vi "DAQ_Main.vi"() -> ()   [LabVIEW 2026]
panel:
  out "samples_logged":dbl
  out "overpressure":bool
  out "pressure_chart":dbl(graph)
  out "pressure_bar":dbl
  in  "stop_acquisition":bool
  in  "start_acquisition":bool
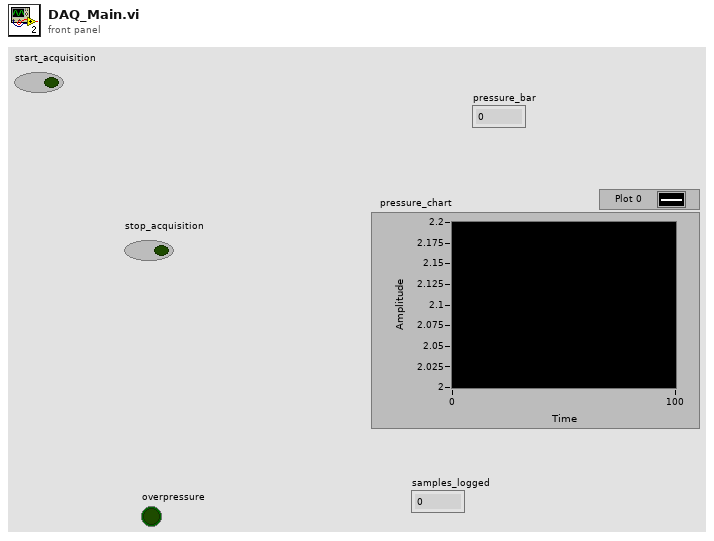
[diagram p1: front panel]
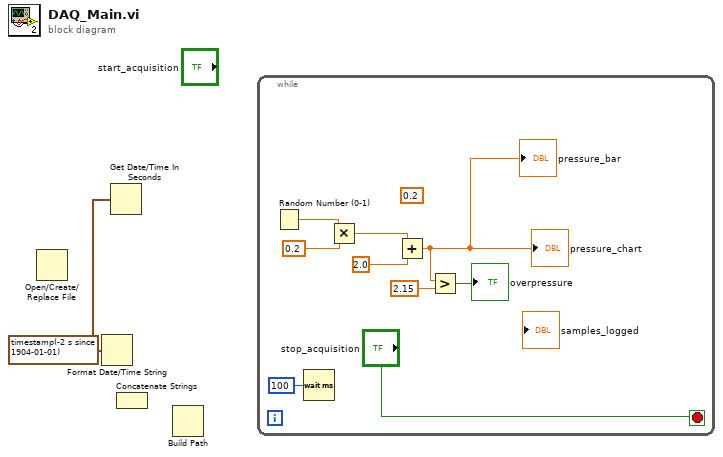
[diagram p0: block diagram]
diagram:
  (unwired) timestamp(-2 s since 1904-01-01) ("time stamp")
  n1 = Open/Create/Replace File() -> ()  [unwired: 6 in, 3 out]
  n2 = Get Date/Time In Seconds() -> (seconds since 1Jan1904=w1:timestamp)
  n3 = Format Date/Time String(seconds (now)=w1) -> ()  [unwired: 2 in, 1 out]
  n4 = Concatenate Strings() -> ()  [unwired: 2 in, 1 out]
  n5 = Build Path() -> ()  [unwired: 2 in, 1 out]
  n6 = while {
    stop <- "stop_acquisition" stop-if-true
    (unwired) 0.2 ("x*y")
    n7 = Random Number (0-1)() -> (number: 0 to 1=w8:dbl)
    n8 = Wait (ms)(milliseconds to wait=u32 100) -> ()  [unwired: 1 out]
    n9 = Multiply(x=w8, y=0.2 ("x*y")) -> (x*y=w6:dbl)
    n10 = Add(x=w6, y=2.0) -> (x+y=w4:dbl)
    "pressure_bar" <- w4
    "pressure_chart" <- w4
    n11 = Greater?(x=w4, y=2.15) -> (0:→"overpressure":bool)
  }
